vi "Red--constant.vi"() -> (1 "Red":u32(colorbox))   [LabVIEW 2018, in "Band Colors.lvlib"]
doc: "Provides the RGB color value for red.\n\nThe VI converts the RGB components (220, 0, 0) into a LabVIEW color value and returns it through <b>Red</b>."
uses:
  Band Colors.lvlib
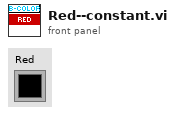
[diagram p1: front panel]
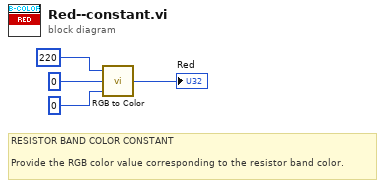
[diagram p0: block diagram]
diagram:
  # "RESISTOR BAND COLOR CONSTANT\n\nProvide the RGB color value corresponding to the resistor band color."
  n1 = call <vilib>:"RGB to Color.vi"("B"=u8 0, "G"=u8 0, "R"=u8 220) -> ("Color"=→"Red":u32)
